vi "Calling Class Methods.vi"() -> ()   [LabVIEW 2020]
uses:
  688a6956-cd2d-4b8a-a8be-e172edc5432f.vi
  2e819b81-fe13-4050-befc-599fc726c07c.vi
  688a6956-cd2d-4b8a-a8be-e172edc5432f.vi/6c7a13f1-33d3-431d-8188-904cac5422b3.vi
  G-Embedded-Python-Interpreter-Toolkit/Python Object Reference to Pointer Sized Ref.vi
  2e819b81-fe13-4050-befc-599fc726c07c.vi/6c7a13f1-33d3-431d-8188-904cac5422b3.vi
  G-Embedded-Python-Interpreter-Toolkit/Pointer Sized Ref to Python Object Reference.vi
  G-Embedded-Python-Interpreter-Toolkit/Merge Call Library Errors.vi
  G-Embedded-Python-Interpreter-Toolkit/Generate Argument Type Info.vi
  G-Embedded-Python-Interpreter-Toolkit/G-Embedded-Python-Interpreter-Toolkit.lvlib
  6d5f1638-640c-4e20-b011-0cee3ae60b95.vi
panel:
  in  "Decrement":bool
  in  "Increment":bool
  out "Counter Value":i32 format="%011d"
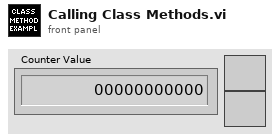
[diagram p1: front panel]
types:
  T1 = typedef "G-Embedded-Python-Interpreter-Toolkit.lvlib/Python Object Reference.ctl" = refnum<k1>
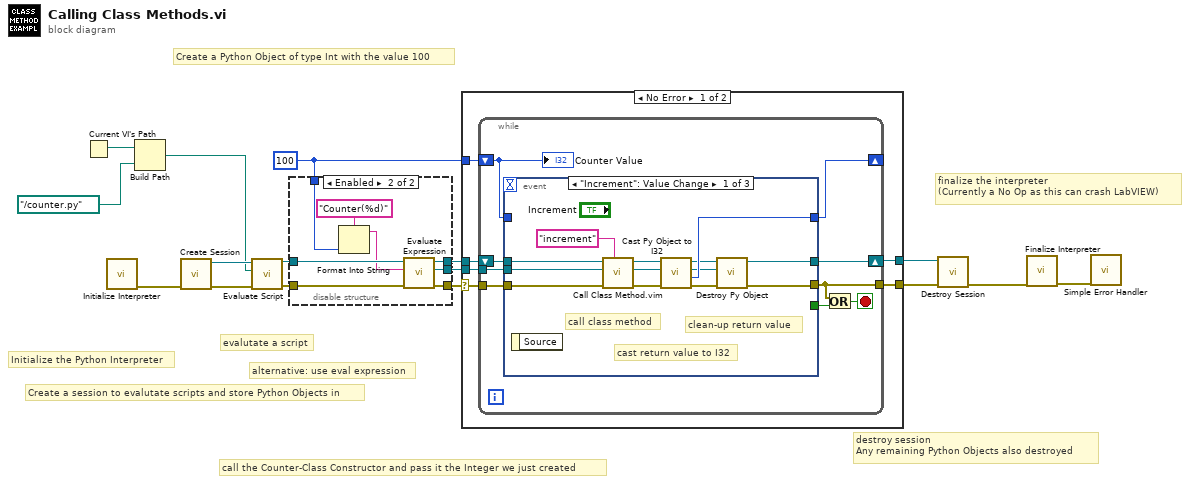
[diagram p0: block diagram]
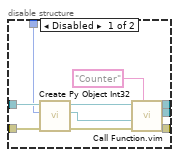
[diagram p2: hidden frame]
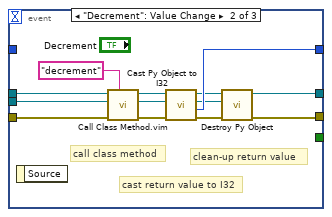
[diagram p3: hidden frame]
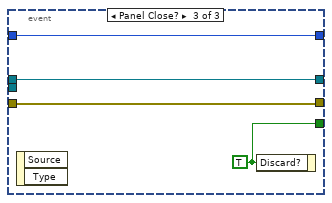
[diagram p4: hidden frame]
diagram:
  w8 = 100 ("Value")
  # "alternative: use eval expression"
  # "finalize the interpreter\n(Currently a No Op as this can crash LabVIEW)"
  # "destroy session \nAny remaining Python Objects also destroyed"
  # "Create a Python Object of type Int with the value 100"
  # "call the Counter-Class Constructor and pass it the Integer we just created"
  # "evalutate a script"
  # "Create a session to evalutate scripts and store Python Objects in"
  # "Initialize the Python Interpreter"
  n1 = Current VI's Path() -> (path=w13:path)
  n2 = call "Initialize Interpreter.vi"() -> ("error out"=w16:errorcluster)  [unwired: 10 in, 1 out]
  n3 = Build Path(base path=w13, name or relative path=path "../counter.py") -> (appended path=w11:path)
  n4 = call "Create Session.vi"("error in (no error)"=w16) -> ("error out"=w15:errorcluster, "Session Handle"=w14:refnum<data-value>)  [unwired: 9 in]
  n5 = call "Evaluate Script.vi"("error in (no error)"=w15, "Script File Path"=w11, "Session Handle in"=w14) -> ("error out"=w9:errorcluster, "Session Handle out"=w10:refnum<data-value>)  [unwired: 7 in]
  n6 = disable-structure shown="Enabled" {
    disable-tunnel: w10 -> [w25 w34]
    disable-tunnel: w9 -> [w24 w33]
    disable-tunnel: w8 -> [w21 w29]
    disable-tunnel: [w20 w32] -> w7
    disable-tunnel: [w19 w31] -> w6
    disable-tunnel: [w18 w30] -> w5
    frame Disabled {
      n7 = call "Create Py Object Int32.vi"("error in (no error)"=w24, "Value"=w21, "Session Handle in"=w25) -> ("error out"=w23:errorcluster, "Python Object Refnum"=w17:T1, "Session Handle out"=w22:refnum<data-value>)  [unwired: 6 in]
      n8 = call "Call Function.vim"("Function Name"="Counter", "error in (no error)"=w23, "Arguments in (Default - None)"=w17, "Data Value Reference in"=w22) -> ("error out"=w20:errorcluster, "Returned Python Object Refnum"=w18:T1, "Data Value Reference out"=w19:refnum<data-value>)  [unwired: 5 in]
    }
    frame Enabled {
      n9 = Format Into String(format string="Counter(%d)", w29) -> (resulting string=w27:string)  [unwired: 2 in, 1 out]
      n10 = call "Evaluate Expression.vi"("error in (no error)"=w33, "Expression"=w27, "Session Handle in"=w34) -> ("error out"=w32:errorcluster, "Python Object Refnum"=w30:T1, "Session Handle out"=w31:refnum<data-value>)  [unwired: 6 in]
    }
  }
  n11 = case shown="No Error" w7 {
    selector: w7 -> [w39 w81]
    tunnel: w8 -> [w40 _]
    tunnel: w6 -> [w38 w80]
    tunnel: w5 -> [w37 _]
    tunnel: [w36 w81] -> w4
    tunnel: [w35 w80] -> w3
    frame No Error {
      n12 = while {
        tunnel: w39 -> [w49]
        shift-right: [w44] -> w35
        shift-left: w38 -> [w48]
        tunnel: w37 -> [w47]
        shift-right: [w46] -> _
        shift-left: w40 -> [w43]
        tunnel: [w41] -> w36
        stop <- w45 stop-if-true
        n13 = event shown="[0] \"Increment\": Value Change" {
          selector: _ -> [_ _ _]
          dyn-events: _ -> [_ _ _]
          timeout: _ -> [_ _ _]
          tunnel: w49 -> [w62 w75 w79]
          tunnel: w48 -> [w61 w74 w78]
          tunnel: w47 -> [w60 w73 _]
          tunnel: [w55 w68 w77] -> w46
          tunnel: [w51 w64 w79] -> w41
          tunnel: [w50 w63 w78] -> w44
          tunnel: w43 -> [_ _ w77]
          tunnel: [_ _ w76] -> w42
          event "Increment": Value Change {
            # "clean-up return value"
            # "cast return value to I32"
            # "call class method"
            n14 = event-data() -> ()  [unwired: 1 in, 1 out]
            n15 = call "Call Class Method.vim"("Function Name"="increment", "error in (no error)"=w62, "Class Instance"=w60, "Data Value Reference in"=w61) -> ("error out"=w58:errorcluster, "Returned Python Object Refnum"=w56:T1, "Data Value Reference out"=w57:refnum<data-value>)  [unwired: 5 in]
            n16 = call "Cast Py Object to I32.vi"("error in (no error)"=w58, "Python Object Refnum in"=w56, "Session Handle in"=w57) -> ("error out"=w52:errorcluster, "Value"=w55:i32, "Python Object Refnum out"=w53:T1, "Session Handle out"=w54:refnum<data-value>)  [unwired: 5 in]
            n17 = call "Destroy Py Object.vi"("error in (no error)"=w52, "Python Object Refnum"=w53, "Session Handle in"=w54) -> ("error out"=w51:errorcluster, "Session Handle out"=w50:refnum<data-value>)  [unwired: 7 in]
          }
          event "Decrement": Value Change {
            # "clean-up return value"
            # "cast return value to I32"
            # "call class method"
            n18 = event-data() -> ()  [unwired: 1 in, 1 out]
            n19 = call "Call Class Method.vim"("Function Name"="decrement", "error in (no error)"=w75, "Class Instance"=w73, "Data Value Reference in"=w74) -> ("error out"=w71:errorcluster, "Returned Python Object Refnum"=w69:T1, "Data Value Reference out"=w70:refnum<data-value>)  [unwired: 5 in]
            n20 = call "Cast Py Object to I32.vi"("error in (no error)"=w71, "Python Object Refnum in"=w69, "Session Handle in"=w70) -> ("error out"=w65:errorcluster, "Value"=w68:i32, "Python Object Refnum out"=w66:T1, "Session Handle out"=w67:refnum<data-value>)  [unwired: 5 in]
            n21 = call "Destroy Py Object.vi"("error in (no error)"=w65, "Python Object Refnum"=w66, "Session Handle in"=w67) -> ("error out"=w64:errorcluster, "Session Handle out"=w63:refnum<data-value>)  [unwired: 7 in]
          }
          event Panel Close? {
            w76 = TRUE ("Discard?")
            n22 = event-data() -> ()  [unwired: 1 in, 2 out]
            n23 = event-data("Discard?"=w76) -> ()  [unwired: 1 in, 1 out]
          }
        }
        n24 = Or(x=w41, y=w42) -> (x .or. y?=w45:bool)
        "Counter Value" <- w43
      }
    }
    frame Error {
    }
  }
  n25 = call "Destroy Session.vi"("error in (no error)"=w4, "Session Handle"=w3) -> ("error out"=w2:errorcluster)  [unwired: 9 in]
  n26 = call "Finalize Interpreter.vi"("error in (no error)"=w2) -> ("error out"=w1:errorcluster)  [unwired: 10 in]
  n27 = call <vilib>:"Simple Error Handler.vi"("error in (no error)"=w1) -> ()  [unwired: 4 in, 5 out]
